vi "Sort an Array.vi"() -> ()   [LabVIEW 2026]
panel:
  out "Sorted Array":dbl[](array[numeric])
  in  "Sorting Order":enum16{"Ascending Order", "Descending Order"}(ring)
  in  "Input Array":dbl[](array[numeric])
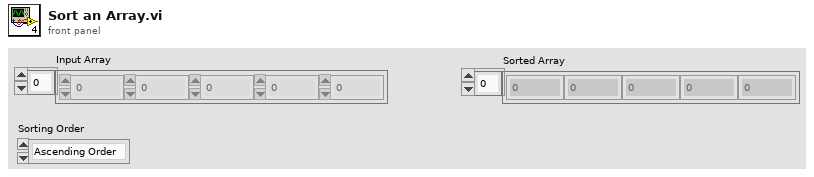
[diagram p1: front panel]
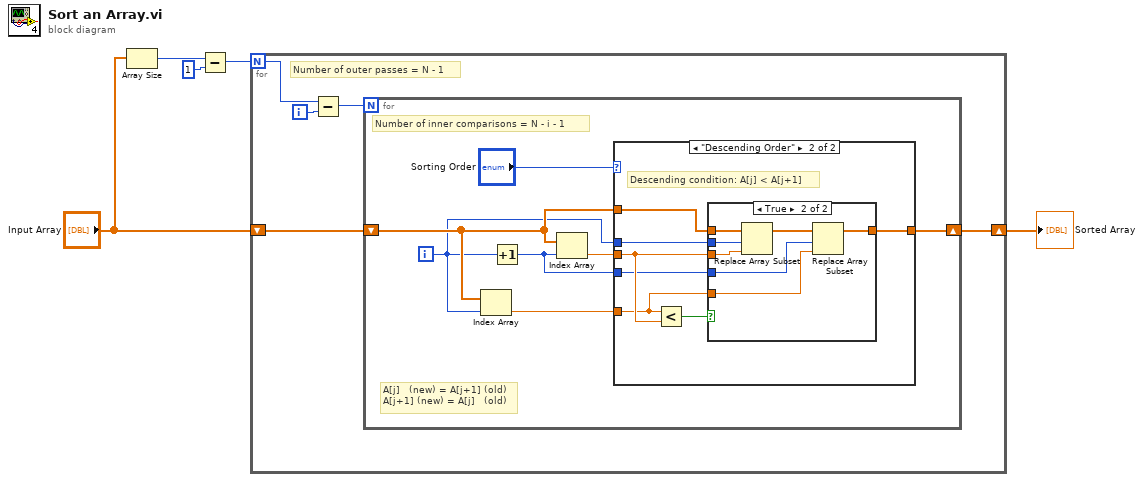
[diagram p0: block diagram]
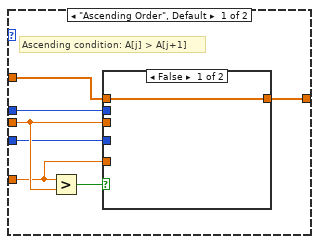
[diagram p2: hidden frame]
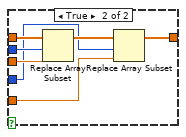
[diagram p3: hidden frame]
diagram:
  n1 = Array Size(array="Input Array") -> (size(s)=w5:i32)
  n2 = Subtract(x=w5, y=1) -> (x-y=w3:i32)
  n3 = for {
    N: w3 -> [w9]
    shift-right: [w6] -> w1
    shift-left: "Input Array" -> [w7]
    i -> [w8]
    # "Number of outer passes = N - 1"
    n4 = Subtract(x=w9, y=w8) -> (x-y=w10:i32)
    n5 = for {
      N: w10 -> [_]
      shift-right: [w11] -> w6
      shift-left: w7 -> [w15]
      i -> [w14]
      # "A[j]   (new) = A[j+1] (old)\nA[j+1] (new) = A[j]   (old)"
      # "Number of inner comparisons = N - i - 1"
      n6 = Index Array(array=w15, index=w14) -> (element=w12:dbl)
      n7 = Increment(x=w14) -> (x+1=w13:i32)
      n8 = Index Array(array=w15, index=w13) -> (element=w16:dbl)
      n9 = case shown="\"Descending Order\"" "Sorting Order" {
        tunnel: w12 -> [w19 w34]
        tunnel: w16 -> [w21 w36]
        tunnel: w15 -> [w23 w38]
        tunnel: w14 -> [w22 w37]
        tunnel: w13 -> [w20 w35]
        tunnel: [w18 w33] -> w11
        frame "Ascending Order", Default {
          # "Ascending condition: A[j] > A[j+1]"
          n10 = Greater?(x=w19, y=w21) -> (0:w24:bool)
          n11 = case shown="False" w24 {
            tunnel: w23 -> [w25 w32]
            tunnel: w22 -> [_ w31]
            tunnel: w21 -> [_ w30]
            tunnel: w20 -> [_ w28]
            tunnel: w19 -> [_ w27]
            tunnel: [w25 w26] -> w18
            frame False {
            }
            frame True {
              n12 = Replace Array Subset(array=w32, new element=w30, index=w31) -> (w29:dbl[])
              n13 = Replace Array Subset(array=w29, new element=w27, index=w28) -> (w26:dbl[])
            }
          }
        }
        frame "Descending Order" {
          # "Descending condition: A[j] < A[j+1]"
          n14 = Less?(x=w34, y=w36) -> (x < y?=w39:bool)
          n15 = case shown="True" w39 {
            tunnel: w38 -> [w40 w47]
            tunnel: w37 -> [_ w46]
            tunnel: w36 -> [_ w45]
            tunnel: w35 -> [_ w43]
            tunnel: w34 -> [_ w42]
            tunnel: [w40 w41] -> w33
            frame False {
            }
            frame True {
              n16 = Replace Array Subset(array=w47, new element=w45, index=w46) -> (w44:dbl[])
              n17 = Replace Array Subset(array=w44, new element=w42, index=w43) -> (w41:dbl[])
            }
          }
        }
      }
    }
  }
  "Sorted Array" <- w1
